vi "ZM-CP-UDP-receive.vi"(8 "error in (no error)":errorcluster, 10 "timeout_ms":i32, 11 "ZM-CP-UDP-receiver in":refnum<class "ZM-CP-UDP-receiver.lvclass">) -> (0 "error out":errorcluster, 1 "timed_out":bool, 2 "json":string, 3 "ZM-CP-UDP-receiver out":refnum<class "ZM-CP-UDP-receiver.lvclass">)   [LabVIEW 2020, in "ZM-CP-UDP-udp_transport.lvlib" / "ZM-CP-UDP-receiver.lvclass"]
doc: "Reads one datagram (one JSON line) from the UDP receiver, waiting up to timeout_ms. A timeout is not an error: it returns timed_out = TRUE and an empty json. Every other error passes on."
uses:
  ZM-CP-UDP-receiver.lvclass
  ZM-CP-UDP-receiver.lvclass/ZM-CP-UDP-receiver.ctl
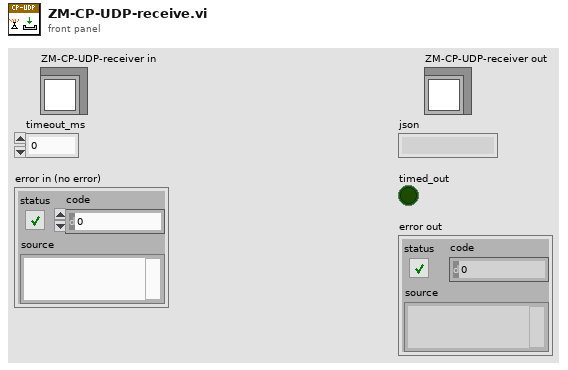
[diagram p1: front panel]
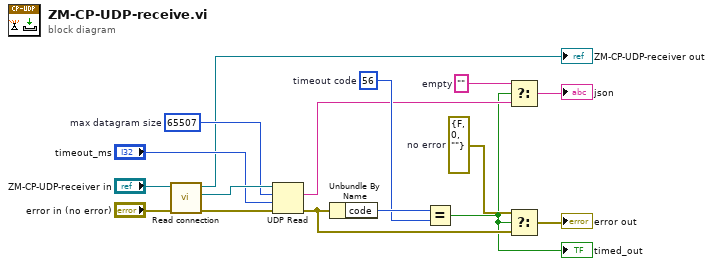
[diagram p0: block diagram]
diagram:
  w6 = ""  # empty
  w8 = errorcluster {"status"=FALSE, "code"=0, "source"=""}  # no error
  w9 = 56  # timeout code
  w13 = 65507  # max datagram size
  n1 = call "Read connection.vi"("error in (no error)"="error in (no error)", "ZM-CP-UDP-receiver in"="ZM-CP-UDP-receiver in") -> ("error out"=w11:errorcluster, "connection"=w14:refnum<k16>, "ZM-CP-UDP-receiver out"=→"ZM-CP-UDP-receiver out":refnum<class "ZM-CP-UDP-receiver.lvclass">)  [unwired: 7 in]
  n2 = UDP Read(connection ID=w14, max size (548)=w13, timeout ms (25000)="timeout_ms", 8:w11) -> (data out=w5:string, error out=w7:errorcluster)  [unwired: 3 out]
  n3 = Unbundle By Name(w7) -> ("code"=w10:i32)
  n4 = Equal?(x=w10, y=w9) -> (x = y?=w2:bool)
  "timed_out" <- w2
  n5 = Select(t=w6, s=w2, f=w5) -> (s? t:f=→"json":string)
  n6 = Select(t=w8, s=w2, f=w7) -> (s? t:f=→"error out":errorcluster)
